vi "PID Parameters.vi"(8 "error in (no error)":errorcluster, 11 "Node Ptr":T1 format="%.0x") -> (0 "error out":errorcluster)   [LabVIEW 2019, in "Control Addon System Explorer.lvlib"]
uses:
  Control Addon System Explorer.lvlib
  <vilib>/NI VeriStand/Custom Device API/Custom Device Item Ref.ctl
  NationalInstruments.VeriStand.SystemStorageUI
  Types/Action.ctl
  Addon Shared/SubVIs/Constants.vi
  <vilib>/NI VeriStand/Custom Device API/NI VeriStand - Get Item Property.vi
  <vilib>/NI VeriStand/Custom Device API/Get Item Property (Boolean).vi
  <vilib>/NI VeriStand/Custom Device API/Get Item Property (String).vi
  <vilib>/NI VeriStand/Custom Device API/NI VeriStand - Set Item Property.vi
  <vilib>/NI VeriStand/Custom Device API/Set Item Property (Boolean).vi
  <vilib>/NI VeriStand/Custom Device API/Set Item Property (String).vi
  <vilib>/NI VeriStand/UI Controls/Single Node Browser/Register Callbacks.vi
  <vilib>/NI VeriStand/Custom Device API/Custom Device API.lvlib
  Addon Shared/Control Addon Shared.lvlib
panel:
  in  "Export":bool
  in  "Import":bool
  in  "Reset":bool
  in  "Apply":bool
  in  "Header 3":cluster{"Section Name":string}={"Section Name"="Gain Settings"}
  in  "Enable Live Updates":bool
  in  "PID Settings":i32(listbox)
  in  "Gain Schedule Channel":refnum<k24>(container) caption="Gain Schedule Signal"
  in  "Header 2":cluster{"Section Name":string}={"Section Name"="Gain Schedule Settings"}
  in  "Enable Gain Scheduling":bool
  in  "SHDocVw.IWebBrowser":refnum<k7>(container)
  in  "Header":cluster{"Section Name":string}={"Section Name"="Parameters Settings"}
  in  "Description":string
  out "Name":string
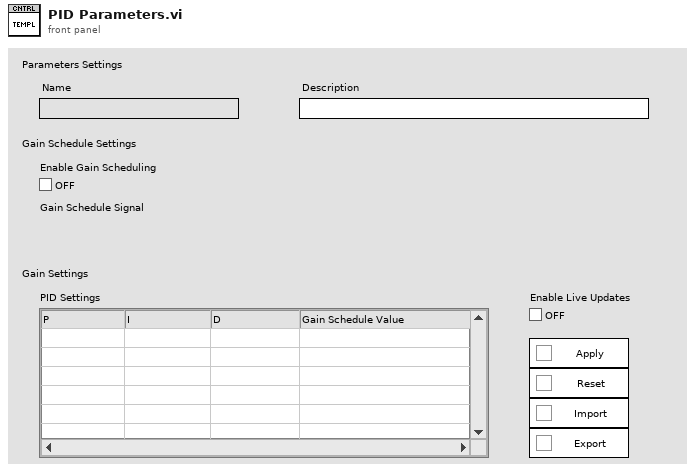
[diagram p1: front panel]
types:
  T1 = typedef "Custom Device API.lvlib/Custom Device Item Ref.ctl" = u64
  T2 = typedef "Control Addon System Explorer.lvlib/Action.ctl" = enum16{"Get", "Set"}
  T3 = typedef "Control Addon Shared.lvlib/PID Parameters.ctl" = cluster{"Enable Live Updates":bool, "Enable Gain Scheduling":bool, "PID Parameters":dbl[][]}
  T4 = typedef "Control Addon System Explorer.lvlib/PID Parameters Channel Browser Refs.ctl" = cluster{"GainSchedule":refnum<user-event>}
  T5 = typedef "Custom Device API.lvlib/Custom Device Item Info.ctl" = cluster{"Name":string, "Is Channel":bool, "GUID":string, "Is Waveform":bool}
  T6 = typedef "Custom Device API.lvlib/Custom Device Commands.ctl" = enum16{"Default", "Item renamed", "Shutdown", "Dynamic button pressed"}
  T7 = typedef "LVPoint32TypeDef.ctl" = cluster{"Horizontal":i32, "Vertical":i32}
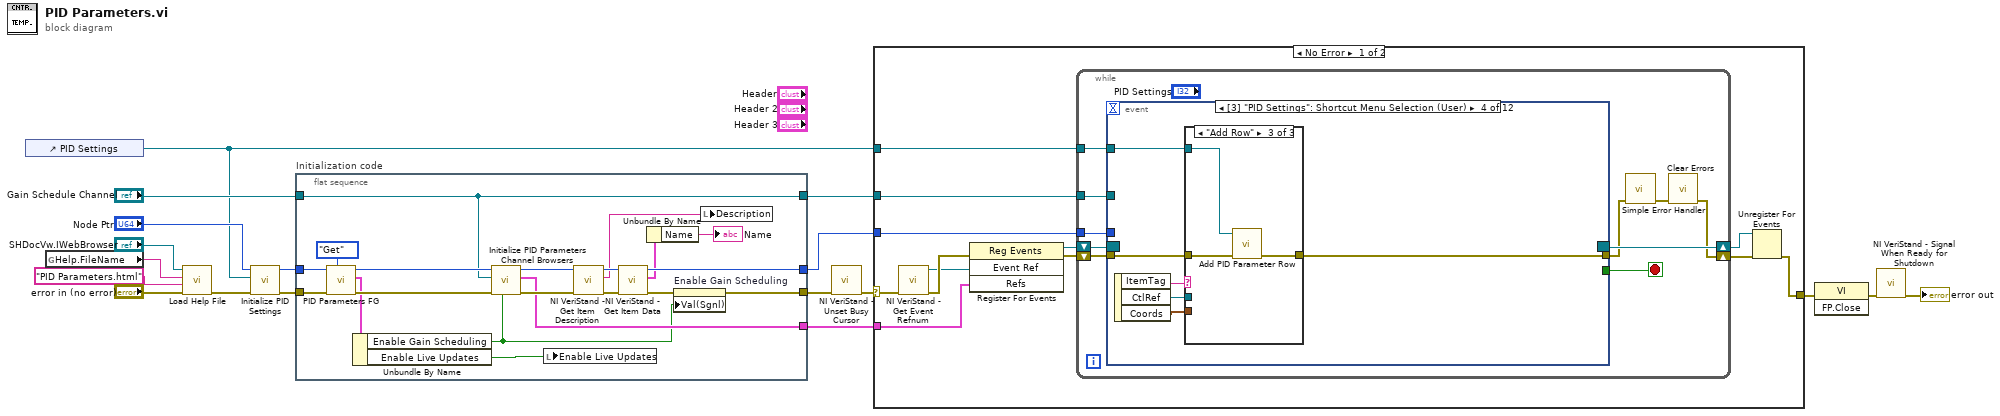
[diagram p0: block diagram]
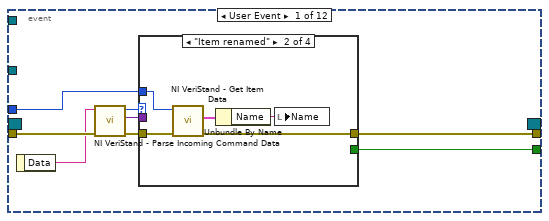
[diagram p2: hidden frame]
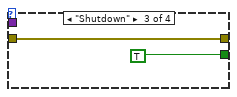
[diagram p4: hidden frame]
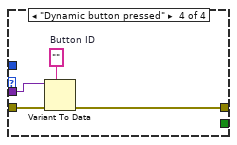
[diagram p5: hidden frame]
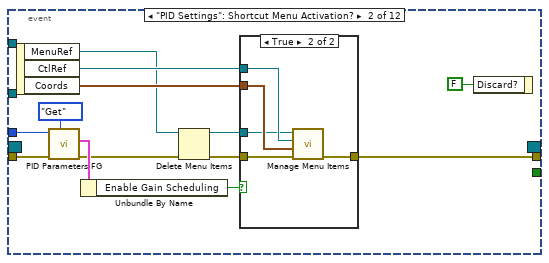
[diagram p6: hidden frame]
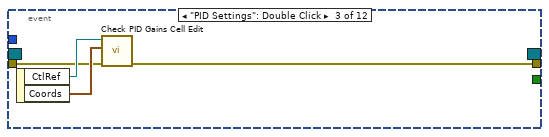
[diagram p8: hidden frame]
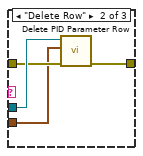
[diagram p10: hidden frame]
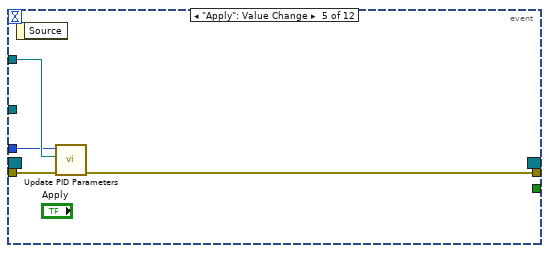
[diagram p11: hidden frame]
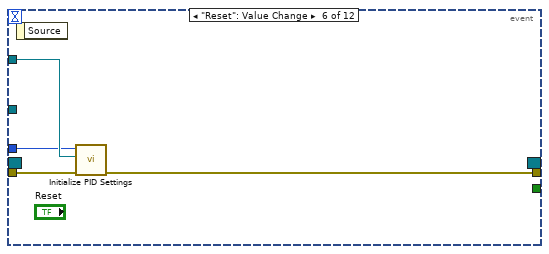
[diagram p12: hidden frame]
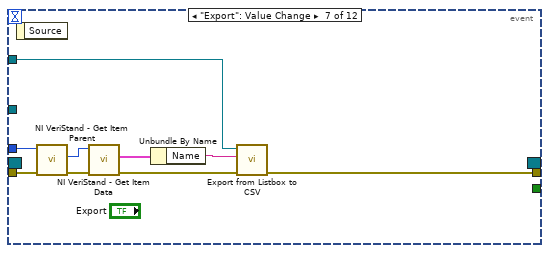
[diagram p13: hidden frame]
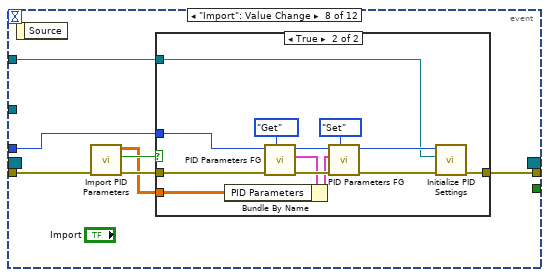
[diagram p14: hidden frame]
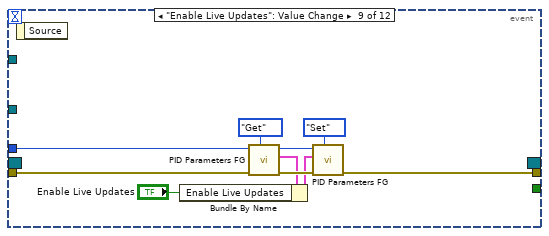
[diagram p16: hidden frame]
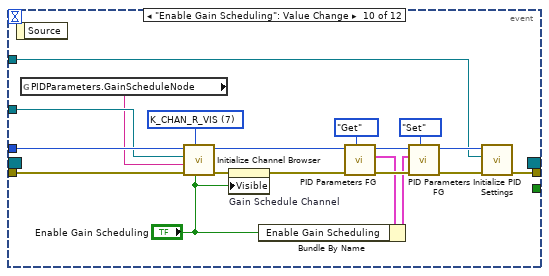
[diagram p17: hidden frame]
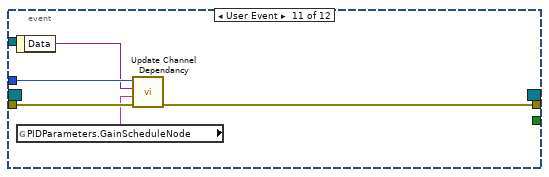
[diagram p18: hidden frame]
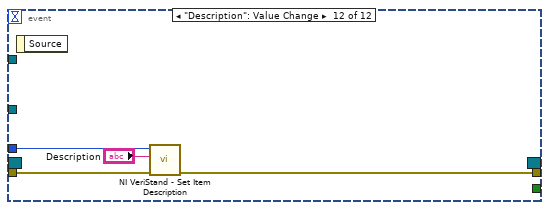
[diagram p19: hidden frame]
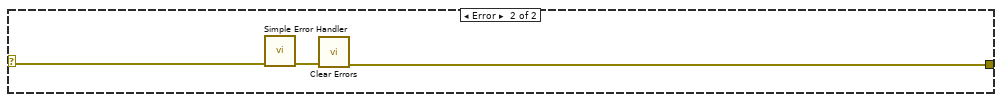
[diagram p20: hidden frame]
diagram:
  n1 = control-ref of="PID Settings"() -> (w3:refnum<vi>)
  n2 = global read "Constants.vi" "Help.FileName"() -> (w1:string)
  n3 = call "Load Help File.vi"("error in (no error)"="error in (no error)", "HTML File"="PID Parameters.html", "Main CHM File"=w1, "SHDocVw.IWebBrowser2"="SHDocVw.IWebBrowser") -> ("error out"=w7:errorcluster)  [unwired: 7 in]
  n4 = call "Initialize PID Settings.vi"("error in (no error)"=w7, "PID Settings"=w3, "Item Ref in"="Node Ptr") -> ("error out"=w6:errorcluster, "Item Ref out"=w4:T1)  [unwired: 7 in]
  n5 = flat-sequence "Initialization code" {
    tunnel: w6 -> [w32]
    tunnel: w4 -> [w30]
    tunnel: [w23] -> w15
    tunnel: [w38] -> w13
    tunnel: "Gain Schedule Channel" -> [w19]
    tunnel: [w25] -> w8
    tunnel: [w19] -> w2
    frame #0 {
      n6 = call "PID Parameters FG.vi"("Action"=Action."Get", "error in (no error)"=w32, "Node Ptr"=w30) -> ("error out"=w31:errorcluster, "Parameters"=w28:T3, "Item Ref out"=w22:T1)  [unwired: 6 in]
      n7 = Unbundle By Name(w28) -> ("Enable Gain Scheduling"=w21:bool, "Enable Live Updates"=w27:bool)
      n8 = call "Initialize PID Parameters Channel Browsers.vi"("Enable Gain Scheduling"=w21, "error in (no error)"=w31, "Channel Browser"=w19, "Item Ref in"=w22) -> ("error out"=w26:errorcluster, "Refs"=w25:T4, "Item Ref out"=w20:T1)  [unwired: 5 in]
      n9 = local write "Enable Live Updates"(w27) -> ()
      n10 = call <vilib>:"NI VeriStand - Get Item Description.vi"("error in (no error)"=w26, "Item Ref in"=w20) -> ("error out"=w35:errorcluster, "Description"=w36:string, "Item Ref out"=w37:T1)  [unwired: 7 out]
      n11 = call <vilib>:"NI VeriStand - Get Item Data.vi"("error in (no error)"=w35, "Item Ref in"=w37) -> ("error out"=w24:errorcluster, "Item Info"=w34:T5, "Item Ref out"=w38:T1)  [unwired: 7 out]
      n12 = Unbundle By Name(w34) -> ("Name"=→"Name":string)
      n13 = property on="Enable Gain Scheduling" class="Bool (strict)"(error in=w24, "Val(Sgnl)"=w21) -> (error out=w23:errorcluster)  [unwired: 1 in, 1 out]
      n14 = local write "Description"(w36) -> ()
    }
  }
  n15 = call <vilib>:"NI VeriStand - Unset Busy Cursor.vi"("error in (no error)"=w15) -> ("error out"=w14:errorcluster)  [unwired: 10 out]
  n16 = case shown="No Error" w14 {
    selector: w14 -> [w42 w196]
    tunnel: [w47 w194] -> w18
    tunnel: w13 -> [w43 _]
    tunnel: w8 -> [w41 _]
    tunnel: w3 -> [w40 _]
    tunnel: w2 -> [w39 _]
    frame No Error {
      n17 = call <vilib>:"NI VeriStand - Get Event Refnum.vi"("error in (no error)"=w42) -> ("error out"=w50:errorcluster, "Event Ref"=w46:refnum<user-event>)  [unwired: 9 out]
      n18 = register-events(error in=w50, w46, w41) -> (reference out=w44:refnum<event-registration>, error out=w45:errorcluster)  [unwired: 1 in]
      n19 = while {
        tunnel: w43 -> [w56]
        shift-right: [w53] -> w48
        shift-left: w45 -> [w59]
        shift-right: [w60] -> w49
        shift-left: w44 -> [w58]
        tunnel: w40 -> [w52]
        tunnel: w39 -> [w51]
        stop <- w57 stop-if-true
        n20 = event shown="[3] \"PID Settings\": Shortcut Menu Selection (User)" {
          selector: w58 -> [_ _ _ _ _ _ _ _ _ _ _ _]
          dyn-events: [_ _ _ _ _ _ _ _ _ _ _ _] -> w60
          timeout: _ -> [_ _ _ _ _ _ _ _ _ _ _ _]
          tunnel: w59 -> [w68 w88 w101 w109 w121 w125 w132 w141 w164 w176 w189 w192]
          tunnel: [w64 _ _ _ _ _ _ _ _ _ _ _] -> w57
          tunnel: [w63 w90 w100 w106 w120 w122 w133 w139 w156 w168 w185 w191] -> w55
          tunnel: w56 -> [w62 w87 _ _ w118 w123 w134 w136 w163 w174 w188 w193]
          tunnel: w52 -> [_ _ _ w107 w119 w124 w126 w135 _ w166 _ _]
          tunnel: w51 -> [_ _ _ _ _ _ _ _ _ w171 _ _]
          event User Event {
            n21 = event-data() -> ("Data"=w67:string)  [unwired: 1 out]
            n22 = call <vilib>:"NI VeriStand - Parse Incoming Command Data.vi"("error in (no error)"=w68, "Incoming data"=w67) -> ("error out"=w66:errorcluster, "Outgoing data"=w61:variant, "Action"=w65:T6)  [unwired: 7 out]
            n23 = case shown="\"Item renamed\"" w65 {
              tunnel: w66 -> [w69 w74 w75 w80]
              tunnel: [_ _ TRUE _] -> w64
              tunnel: [w69 w71 w75 w77] -> w63
              tunnel: w62 -> [_ w73 _ _]
              tunnel: w61 -> [_ _ _ w79]
              frame "Default", Default {
              }
              frame "Item renamed" {
                n24 = call <vilib>:"NI VeriStand - Get Item Data.vi"("error in (no error)"=w74, "Item Ref in"=w73) -> ("error out"=w71:errorcluster, "Item Info"=w72:T5)  [unwired: 8 out]
                n25 = Unbundle By Name(w72) -> ("Name"=w70:string)
                n26 = local write "Name"(w70) -> ()
              }
              frame "Shutdown" {
              }
              frame "Dynamic button pressed" {
                w78 = ""  # Button ID
                n27 = Variant To Data(error in=w80, type=w78, Variant=w79) -> (error out=w77:errorcluster)  [unwired: 1 out]
              }
            }
          }
          event "PID Settings": Shortcut Menu Activation? {
            n28 = event-data() -> ("MenuRef"=w82:refnum<k9>, "CtlRef"=w93:refnum<vi>, "Coords"=w92:T7)  [unwired: 1 out]
            n29 = call "PID Parameters FG.vi"("Action"=Action."Get", "error in (no error)"=w88, "Node Ptr"=w87) -> ("error out"=w84:errorcluster, "Parameters"=w86:T3)  [unwired: 6 in, 1 out]
            n30 = Unbundle By Name(w86) -> ("Enable Gain Scheduling"=w85:bool)
            n31 = Delete Menu Items(6:w84, 9:w82) -> (0:w83:errorcluster, 3:w81:refnum<k9>)  [unwired: 2 in]
            n32 = case shown="True" w85 {
              tunnel: w93 -> [_ w99]
              tunnel: w92 -> [_ w98]
              tunnel: w81 -> [_ w97]
              tunnel: [w94 w96] -> w90
              tunnel: w83 -> [w94 w95]
              frame False {
              }
              frame True {
                n33 = call "Manage Menu Items.vi"("error in (no error)"=w95, "Coords"=w98, "CtlRef"=w99, "Menu in"=w97) -> ("error out"=w96:errorcluster)  [unwired: 7 in]
              }
            }
            n34 = event-data("Discard?"=FALSE) -> ()  [unwired: 1 in, 1 out]
          }
          event "PID Settings": Double Click {
            n35 = event-data() -> ("CtlRef"=w103:refnum<vi>, "Coords"=w102:T7)  [unwired: 1 out]
            n36 = call "Check PID Gains Cell Edit.vi"("error in (no error)"=w101, "Coords"=w102, "MulticolumnListbox in"=w103) -> ("error out"=w100:errorcluster)  [unwired: 8 in]
          }
          event "PID Settings": Shortcut Menu Selection (User) {
            n37 = event-data() -> ("ItemTag"=w108:string, "CtlRef"=w105:refnum<vi>, "Coords"=w104:T7)  [unwired: 1 out]
            n38 = case shown="\"Add Row\"" w108 {
              tunnel: w109 -> [w110 w113 w117]
              tunnel: w107 -> [_ _ w116]
              tunnel: [w110 w111 w115] -> w106
              tunnel: w105 -> [_ w114 _]
              tunnel: w104 -> [_ w112 _]
              frame Default {
              }
              frame "Delete Row" {
                n39 = call "Delete PID Parameter Row.vi"("error in (no error)"=w113, "Coords"=w112, "MulticolumnListbox in"=w114) -> ("error out"=w111:errorcluster)  [unwired: 8 in]
              }
              frame "Add Row" {
                n40 = call "Add PID Parameter Row.vi"("error in (no error)"=w117, "MulticolumnListbox in"=w116) -> ("error out"=w115:errorcluster)  [unwired: 9 in]
              }
            }
          }
          event "Apply": Value Change {
            n41 = event-data() -> ()  [unwired: 2 out]
            n42 = call "Update PID Parameters.vi"("error in (no error)"=w121, "PID Settings"=w119, "Item Ref in"=w118) -> ("error out"=w120:errorcluster)  [unwired: 7 in, 1 out]
          }
          event "Reset": Value Change {
            n43 = event-data() -> ()  [unwired: 2 out]
            n44 = call "Initialize PID Settings.vi"("error in (no error)"=w125, "PID Settings"=w124, "Item Ref in"=w123) -> ("error out"=w122:errorcluster)  [unwired: 7 in, 1 out]
          }
          event "Export": Value Change {
            n45 = event-data() -> ()  [unwired: 2 out]
            n46 = call <vilib>:"NI VeriStand - Get Item Parent.vi"("error in (no error)"=w132, "Item Ref in"=w134) -> ("error out"=w130:errorcluster, "Parent Ref"=w131:T1)  [unwired: 6 in, 2 out]
            n47 = call <vilib>:"NI VeriStand - Get Item Data.vi"("error in (no error)"=w130, "Item Ref in"=w131) -> ("error out"=w127:errorcluster, "Item Info"=w129:T5)  [unwired: 8 out]
            n48 = Unbundle By Name(w129) -> ("Name"=w128:string)
            n49 = call "Export from Listbox to CSV.vi"("error in (no error)"=w127, "Name"=w128, "MulticolumnListbox in"=w126) -> ("error out"=w133:errorcluster)  [unwired: 8 in]
          }
          event "Import": Value Change {
            n50 = event-data() -> ()  [unwired: 2 out]
            n51 = call "Import PID Parameters.vi"("error in"=w141) -> ("error out"=w138:errorcluster, "Apply?"=w140:bool, "Parameters"=w137:dbl[][])  [unwired: 8 in]
            n52 = case shown="True" w140 {
              tunnel: [w142 w144] -> w139
              tunnel: w138 -> [w142 w148]
              tunnel: w137 -> [_ w149]
              tunnel: w136 -> [_ w147]
              tunnel: w135 -> [_ w143]
              frame False {
              }
              frame True {
                n53 = call "PID Parameters FG.vi"("Action"=Action."Get", "error in (no error)"=w148, "Node Ptr"=w147) -> ("error out"=w153:errorcluster, "Parameters"=w151:T3, "Item Ref out"=w152:T1)  [unwired: 6 in]
                n54 = Bundle By Name(cluster=w151, "PID Parameters"=w149) -> (w150:T3)
                n55 = call "PID Parameters FG.vi"("Action"=Action."Set", "error in (no error)"=w153, "Parameters"=w150, "Node Ptr"=w152) -> ("error out"=w145:errorcluster, "Item Ref out"=w146:T1)  [unwired: 5 in, 1 out]
                n56 = call "Initialize PID Settings.vi"("error in (no error)"=w145, "PID Settings"=w143, "Item Ref in"=w146) -> ("error out"=w144:errorcluster)  [unwired: 7 in, 1 out]
              }
            }
          }
          event "Enable Live Updates": Value Change {
            n57 = event-data() -> ()  [unwired: 2 out]
            n58 = call "PID Parameters FG.vi"("Action"=Action."Get", "error in (no error)"=w164, "Node Ptr"=w163) -> ("error out"=w161:errorcluster, "Parameters"=w159:T3, "Item Ref out"=w160:T1)  [unwired: 6 in]
            n59 = Bundle By Name(cluster=w159, "Enable Live Updates"="Enable Live Updates") -> (w158:T3)
            n60 = call "PID Parameters FG.vi"("Action"=Action."Set", "error in (no error)"=w161, "Parameters"=w158, "Node Ptr"=w160) -> ("error out"=w156:errorcluster)  [unwired: 5 in, 2 out]
          }
          event "Enable Gain Scheduling": Value Change {
            w177 = u8 7 items=["K_CHAN_R", "K_CHAN_W", "K_CHAN_RW", "K_CHAN_VOLT", "K_CHAN_FAULT", "K_ALL", "K_CUSTOM", "K_CHAN_R_VIS", "K_CHAN_W_VIS", "K_CHAN_RW_VIS", "K_CHAN_VOLT_VIS", "K_CHAN_FAULT_VIS"] ("DisplayFilter")
            n61 = event-data() -> ()  [unwired: 2 out]
            n62 = global read "Constants.vi" "PIDParameters.GainScheduleNode"() -> (w170:string)
            n63 = call "Initialize Channel Browser.vi"("Use Channel?"="Enable Gain Scheduling", "DisplayFilter"=w177, "error in (no error)"=w176, "NodeName"=w170, "Browser Ref"=w171, "Item Ref in"=w174) -> ("error out"=w175:errorcluster, "Item Ref out"=w173:T1)  [unwired: 3 in, 1 out]
            n64 = property on="Gain Schedule Channel" class="AXCont"(error in=w175, "Visible"="Enable Gain Scheduling") -> (error out=w178:errorcluster)  [unwired: 1 in, 1 out]
            n65 = call "PID Parameters FG.vi"("Action"=Action."Get", "error in (no error)"=w178, "Node Ptr"=w173) -> ("error out"=w182:errorcluster, "Parameters"=w180:T3, "Item Ref out"=w181:T1)  [unwired: 6 in]
            n66 = Bundle By Name(cluster=w180, "Enable Gain Scheduling"="Enable Gain Scheduling") -> (w179:T3)
            n67 = call "PID Parameters FG.vi"("Action"=Action."Set", "error in (no error)"=w182, "Parameters"=w179, "Node Ptr"=w181) -> ("error out"=w169:errorcluster, "Item Ref out"=w167:T1)  [unwired: 5 in, 1 out]
            n68 = call "Initialize PID Settings.vi"("error in (no error)"=w169, "PID Settings"=w166, "Item Ref in"=w167) -> ("error out"=w168:errorcluster)  [unwired: 7 in, 1 out]
          }
          event User Event {
            n69 = event-data() -> ("Data"=w187:variant)  [unwired: 1 out]
            n70 = global read "Constants.vi" "PIDParameters.GainScheduleNode"() -> (w186:string)
            n71 = call "Update Channel Dependancy.vi"("error in (no error)"=w189, "NodeName"=w186, "Data"=w187, "Item Ref in"=w188) -> ("error out"=w185:errorcluster)  [unwired: 6 in, 1 out]
          }
          event "Description": Value Change {
            n72 = event-data() -> ()  [unwired: 2 out]
            n73 = call <vilib>:"NI VeriStand - Set Item Description.vi"("error in (no error)"=w192, "Description"="Description", "Item Ref in"=w193) -> ("error out"=w191:errorcluster)  [unwired: 8 out]
          }
        }
        n74 = call <vilib>:"Simple Error Handler.vi"("error in (no error)"=w55) -> ("error out"=w54:errorcluster)  [unwired: 1 in, 7 out]
        n75 = call <vilib>:"Clear Errors.vi"("error in (no error)"=w54) -> ("error out"=w53:errorcluster)  [unwired: 1 in, 5 out]
      }
      n76 = Unregister For Events(event registration refnum=w49, error in=w48) -> (error out=w47:errorcluster)
    }
    frame Error {
      n77 = call <vilib>:"Simple Error Handler.vi"("error in (no error)"=w196) -> ("error out"=w195:errorcluster)  [unwired: 1 in, 7 out]
      n78 = call <vilib>:"Clear Errors.vi"("error in (no error)"=w195) -> ("error out"=w194:errorcluster)  [unwired: 1 in, 5 out]
    }
  }
  n79 = invoke class="VI" method="FP.Close"(error in=w18) -> (error out=w17:errorcluster)  [unwired: 2 in, 2 out]
  n80 = call <vilib>:"NI VeriStand - Signal When Ready for Shutdown.vi"("error in (no error)"=w17) -> ("error out"=→"error out":errorcluster)  [unwired: 10 out]
